vi "From JSON.vi"(8 "error in (no error)":errorcluster, 10 "JSON":string, 11 "Double Float in":refnum<class "Abs_Single Float.lvclass">) -> (0 "error out":errorcluster, 3 "Double Float out":refnum<class "Abs_Single Float.lvclass">)   [LabVIEW 2021, in "Abs_Single Float.lvclass"]
uses:
  Abs_Single Float.lvclass
  Support/Type.ctl
  <vilib>/JDP Science/JSONtext/JSON text to Variant.vi
  <vilib>/JDP Science/JSONtext/LVClass Serializer/JSONtext LVClass Serializer.lvclass
  Abs_Single Float.lvclass/Abs_Single Float.ctl
  Floating Point/Abs_Floating Point.lvclass
  9f794c5c-a91d-4b4c-a4c3-cd9250212edc.vi
  Type/Abs_Type.lvclass
  C:/TSA/LV_Abstract/Source/Abs_Types/Floating Point/Abs_Floating Point.lvclass
  C:/TSA/LV_Abstract/Source/Abs_Types/Numeric/Abs_Numeric.lvclass
  C:/TSA/LV_Abstract/Source/Abs_Types/Value/Abs_Value.lvclass
  C:/TSA/LV_Abstract/Source/Abs_Types/Type/Abs_Type.lvclass
  C:/TSA/LV_Abstract/Source/Abs_Types/Single Float/Abs_Single Float.lvclass
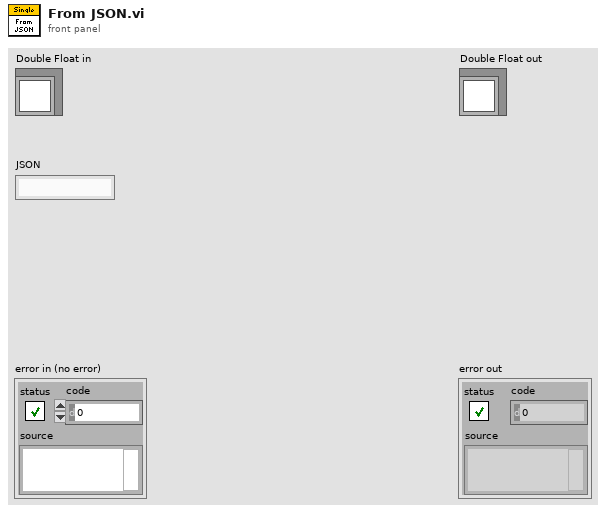
[diagram p1: front panel]
types:
  T1 = typedef "Abs_Single Float.lvclass/Type.ctl" = sgl
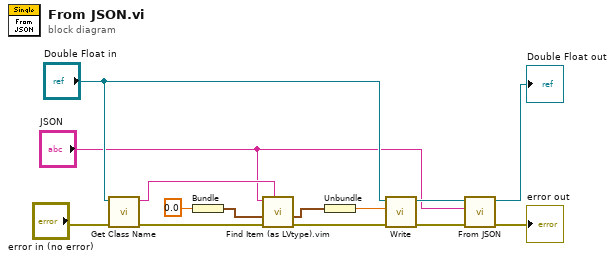
[diagram p0: block diagram]
diagram:
  n1 = call "Get Class Name.vi"("error in (no error)"="error in (no error)", "Abs_Type in"="Double Float in") -> ("error out"=w10:errorcluster, "class name"=w9:string)  [unwired: 8 in]
  n2 = Bundle(T1 0.0) -> (w8:cluster{T1})  [unwired: 1 in]
  n3 = call "Find Item (as LVtype).vim"("$Path or Item Name"=w9, "error in (no error)"=w10, "Data Type and Default Value"=w8, "JSON"="JSON") -> ("error out"=w2:errorcluster, "Data"=w7:cluster{T1})  [unwired: 4 in, 2 out]
  n4 = Unbundle(w7) -> (w3:T1)
  n5 = call-dynamic "Write.vi"("error in (no error)"=w2, "Value"=w3, "Double Float.lvclass_340760 in"="Double Float in") -> ("error out"=w14:errorcluster, "Double Float.lvclass_340760 out"=w13:refnum<class "Abs_Single Float.lvclass">)  [unwired: 7 in]
  n6 = call-parent "From JSON.vi"("error in (no error)"=w14, "JSON"="JSON", "Type in"=w13) -> ("error out"=→"error out":errorcluster, "Type out"=→"Double Float out":refnum<class "Abs_Single Float.lvclass">)  [unwired: 7 in]
